vi "CIF Get Publisher Stats.vi"(8 "error in (no error)":errorcluster, 11 "Publisher Reference":T2) -> (0 "error out":errorcluster, 2 "Last Cnt":u64, 3 "CIF Publisher Stats":T1)   [LabVIEW 2021, in "Iceoryx.lvlib"]
uses:
  Iceoryx.lvlib
  typedef/CIF Pcap Publisher Stats.ctl
  SubVIs/Convert Error Core.vi
  Refnum/Typedef/CIF Publisher Refnum.ctl
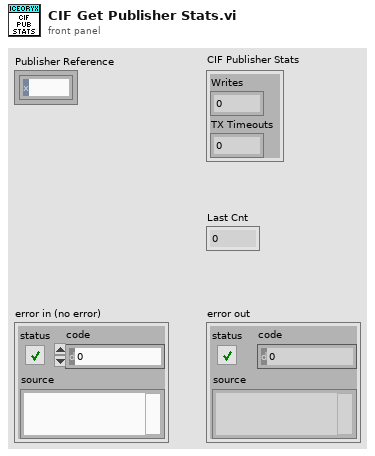
[diagram p1: front panel]
types:
  T1 = typedef "Iceoryx.lvlib/CIF Pcap Publisher Stats.ctl" = cluster{"Writes":u64, "TX Timeouts":u64}
  T2 = typedef "Iceoryx.lvlib/CIF Publisher Refnum.ctl" = refnum<k1>
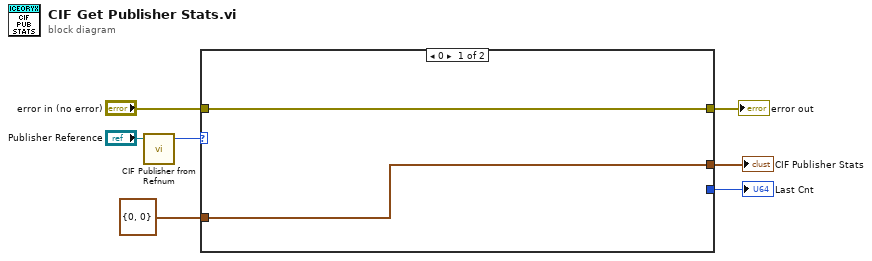
[diagram p0: block diagram]
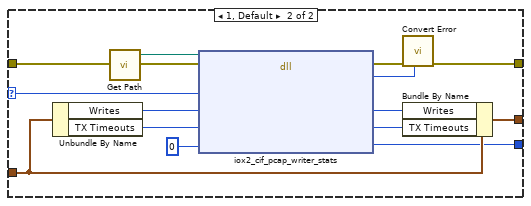
[diagram p2: hidden frame]
diagram:
  n1 = call "CIF Publisher from Refnum.vi"("CIF Publisher Refnum"="Publisher Reference") -> ("CIF Publisher U64"=w1:u64)  [unwired: 4 in]
  n2 = case shown="0" w1 {
    selector: w1 -> [_ w18]
    tunnel: "error in (no error)" -> [w9 w23]
    tunnel: [w9 w19] -> w6
    tunnel: [w8 w14] -> w4
    tunnel: T1 {"Writes"=0, "TX Timeouts"=0} ("CIF Publisher Stats") -> [w8 w11]
    tunnel: [_ w10] -> w2
    frame 0 {
    }
    frame 1, Default {
      n3 = Unbundle By Name(w11) -> ("Writes"=w13:u64, "TX Timeouts"=w12:u64)
      n4 = call "Get Path.vi"() -> ("libiox2_cif path"=w22:path)  [unwired: 4 in]
      n5 = dll-call lib="D:/dev/iceoryx2_lvwrapper/dist/iox2_cif.dll" fn="iox2_cif_pcap_writer_stats"(path in=w22, error in=w23, "writer"=w18, "samples"=w13, "timeouts"=w12, "last_ctr"=u64 0 ("timed_out")) -> (error out=w21:errorcluster, "return type"=w20:i32, "samples"=w15:u64, "timeouts"=w16:u64, "last_ctr"=w10:u64)  [unwired: 2 in, 1 out]
      n6 = call "Convert Error.vi"("return type"=w20, "error in (no error)"=w21) -> ("error out"=w19:errorcluster)  [unwired: 9 in]
      n7 = Bundle By Name(cluster=w11, "Writes"=w15, "TX Timeouts"=w16) -> (w14:T1)
    }
  }
  "error out" <- w6
  "CIF Publisher Stats" <- w4
  "Last Cnt" <- w2
